vi "Save Report to File.vi"(0 "report in":refnum<class "ooWriter.lvclass">, 5 "report file path":path, 7 "prompt to replace? (F)":bool, 9 "password (\"\")":string, 11 "error in (no error)":errorcluster) -> (4 "report out":refnum<class "ooWriter.lvclass">, 15 "error out":errorcluster)   [LabVIEW 2009, in "ooWriter.lvclass"]
doc: "Saves an HTML report to the file specified in <B>report file path</B>. You cannot use this VI with standard reports.\n\nThis VI also saves Microsoft Word and Excel reports."
uses:
  ooWriter.lvclass
  C:/Projets/LAVAG/OpenOfficeRGT/AODL/DLLs/AODL.dll
  ooWriter.lvclass/ooWriter.ctl
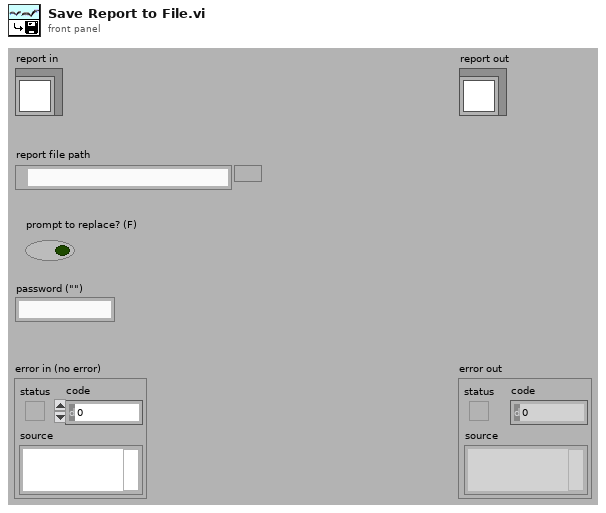
[diagram p1: front panel]
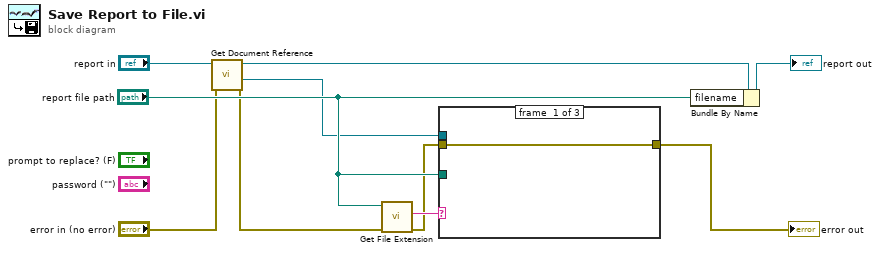
[diagram p0: block diagram]
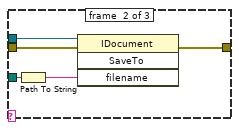
[diagram p2: hidden frame]
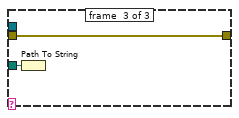
[diagram p3: hidden frame]
diagram:
  n1 = call-dynamic "Get Document Reference.vi"("error in (no error)"="error in (no error)", "ooDocument in"="report in") -> ("error out"=w1:errorcluster, "Document"=w5:refnum<k24>, "ooDocument out"=w3:refnum<class "ooWriter.lvclass">)  [unwired: 7 in]
  n2 = call <vilib>:"Get File Extension.vi"("error in (no error)"=w1, "file"="report file path") -> ("error out"=w6:errorcluster, "lowercase file extension"=w8:string)  [unwired: 6 in, 2 out]
  n3 = case shown="\"odt\"" w8 {
    tunnel: w6 -> [w11 w16 w17]
    tunnel: w5 -> [_ w15 _]
    tunnel: [w11 w13 w17] -> w9
    tunnel: "report file path" -> [_ w12 w18]
    frame #0 {
    }
    frame #1 {
      n4 = Path To String(path=w12) -> (string=w14:string)
      n5 = invoke class="IDocument" method="SaveTo"(reference=w15, error in=w16, "filename"=w14) -> (error out=w13:errorcluster)  [unwired: 1 in, 3 out]
    }
    frame #2 {
      n6 = Path To String(path=w18) -> ()  [unwired: 1 out]
    }
  }
  "error out" <- w9
  n7 = Bundle By Name(cluster=w3, "filename"="report file path") -> (→"report out":refnum<class "ooWriter.lvclass">)
